vi "CE ExNav - VIs Control.vi"(6 "cmd":enum16{"open", "run", "description"}(ring), 8 "error in":errorcluster, 11 "VI path":path) -> (0 "error out":errorcluster, 1 "description":string)   [LabVIEW 2021]
doc: "::: CalcExpress Toolkit :::\nCopyright (c) 2000-2026 Konstantin Shifershteyn. All rights reserved."
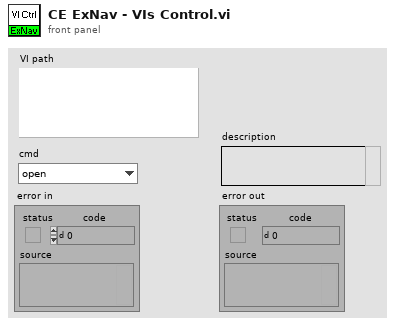
[diagram p1: front panel]
types:
  T1 = enum32{"Invalid", "Standard", "Closed", "Hidden", "Minimized", "Maximized"}
  T2 = enum32{"Bad", "Idle", "Run top level", "Running"}
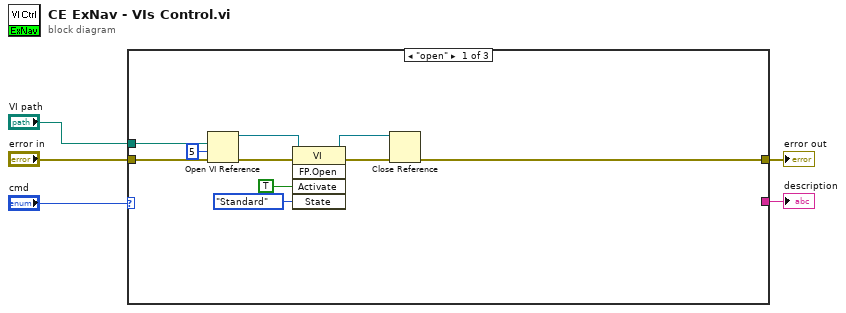
[diagram p0: block diagram]
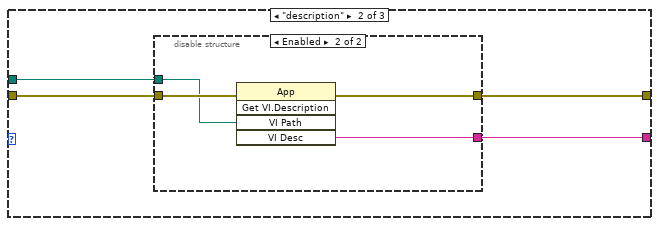
[diagram p2: hidden frame]
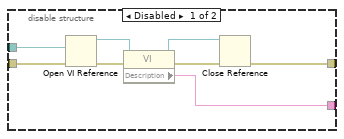
[diagram p3: hidden frame]
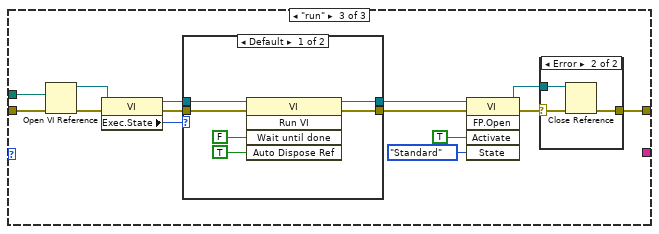
[diagram p4: hidden frame]
diagram:
  n1 = case shown="\"open\"" "cmd" {
    tunnel: "VI path" -> [w9 w19 w45]
    tunnel: "error in" -> [w7 w18 w44]
    tunnel: [w6 w17 w33] -> w2
    tunnel: [_ w16 _] -> w1
    frame "open" {
      n2 = Open VI Reference(vi path=w9, options=5, error in (no error)=w7) -> (vi reference=w12:refnum<vi>, error out=w13:errorcluster)  [unwired: 3 in]
      n3 = invoke class="VI" method="FP.Open"(reference=w12, error in=w13, "Activate"=TRUE ("Activate?"), "State"=T1."Standard") -> (reference out=w10:refnum<vi>, error out=w11:errorcluster)  [unwired: 1 in, 3 out]
      n4 = Close Reference(reference=w10, error in (no error)=w11) -> (error out=w6:errorcluster)
    }
    frame "description" {
      n5 = disable-structure shown="Enabled" {
        disable-tunnel: w19 -> [w23 w29]
        disable-tunnel: w18 -> [w22 w31]
        disable-tunnel: [w21 w30] -> w17
        disable-tunnel: [w20 w28] -> w16
        frame Disabled {
          n6 = Open VI Reference(vi path=w23, error in (no error)=w22) -> (vi reference=w26:refnum<vi>, error out=w27:errorcluster)  [unwired: 4 in]
          n7 = property class="VI"(reference=w26, error in=w27) -> (reference out=w24:refnum<vi>, error out=w25:errorcluster, "Description"=w20:string)
          n8 = Close Reference(reference=w24, error in (no error)=w25) -> (error out=w21:errorcluster)
        }
        frame Enabled {
          n9 = invoke class="App" method="Get VI.Description"(error in=w31, "VI Path"=w29) -> (error out=w30:errorcluster, "VI Desc"=w28:string)  [unwired: 3 in, 3 out]
        }
      }
    }
    frame "run" {
      n10 = Open VI Reference(vi path=w45, error in (no error)=w44) -> (vi reference=w42:refnum<vi>, error out=w43:errorcluster)  [unwired: 4 in]
      n11 = property class="VI"(reference=w42, error in=w43) -> (reference out=w41:refnum<vi>, error out=w39:errorcluster, "Exec.State"=w40:T2)
      n12 = case shown="Default" w40 {
        tunnel: [w52 w57] -> w36
        tunnel: w41 -> [w53 w56]
        tunnel: w39 -> [w51 w57]
        tunnel: [w50 w56] -> w35
        frame Default {
          n13 = invoke class="VI" method="Run VI"(reference=w53, error in=w51, "Wait until done"=FALSE ("Wait Until Done"), "Auto Dispose Ref"=TRUE ("Auto Dispose Reference")) -> (reference out=w50:refnum<vi>, error out=w52:errorcluster)  [unwired: 1 in, 3 out]
        }
        frame "Run top level" {
        }
      }
      n14 = invoke class="VI" method="FP.Open"(reference=w35, error in=w36, "Activate"=TRUE ("Activate?"), "State"=T1."Standard") -> (reference out=w32:refnum<vi>, error out=w34:errorcluster)  [unwired: 1 in, 3 out]
      n15 = case shown="Error" w34 {
        selector: w34 -> [w46 w47]
        tunnel: w32 -> [_ w49]
        tunnel: [w46 w48] -> w33
        frame No Error {
        }
        frame Error {
          n16 = Close Reference(reference=w49, error in (no error)=w47) -> (error out=w48:errorcluster)
        }
      }
    }
  }
  "error out" <- w2
  "description" <- w1
